vi "Periodic Log Filter Check.vi"(0 "Cross CSM Data":T2={"Name (\"\" to Use UUID)"="CSM Tiny", "Current State"="UI: Refresh Buttons", "Arguments"="", "Source Message"={"‘State"="", "’Arguments"="", "’Error"={"status"=FALSE, "code"=0, "source"=""}}, "Source Module"="<end>", "Complete(T)/Start(F)"=TRUE, "LogType"=enum."State Change", "Time Stamp"=timestamp(0 s since 1904-01-01)}, 1 "Reset?":bool, 9 "Remove Immediately? (F)":bool, 11 "Settings":T5={"threashold(#/s)"=2.0, "Check Peroid(s)"=1.0}, 12 "Level (Normal)":T1) -> (4 "Cross CSM Data Out":T2={"Name (\"\" to Use UUID)"="", "Current State"="", "Arguments"="", "Source Message"={"‘State"="", "’Arguments"="", "’Error"={"status"=FALSE, "code"=0, "source"=""}}, "Source Module"="", "Complete(T)/Start(F)"=FALSE, "LogType"=enum."State Change", "Time Stamp"=timestamp(0 s since 1904-01-01)}, 6 "Current Time":timestamp, 10 "Additional Info":string[](array[string]), 14 "Filtered Status":string[](array[string]), 15 "Filtered":bool)   [LabVIEW 2017, in "Communicable State Machine.lvlib" / "LogFilter.lvclass"]
uses:
  LogFilter.lvclass
  Typedef/_CSM_GlobalLog_MSG.ctl
  Typedef/_CSM_Response Source Message.ctl
  Typedef/_CSM_GlobalLog_MSG_TYPE.ctl
  Utility/_support/Periodic String Filter Level.ctl
  Utility/Periodic String Filter State.ctl
  Communicable State Machine.lvlib
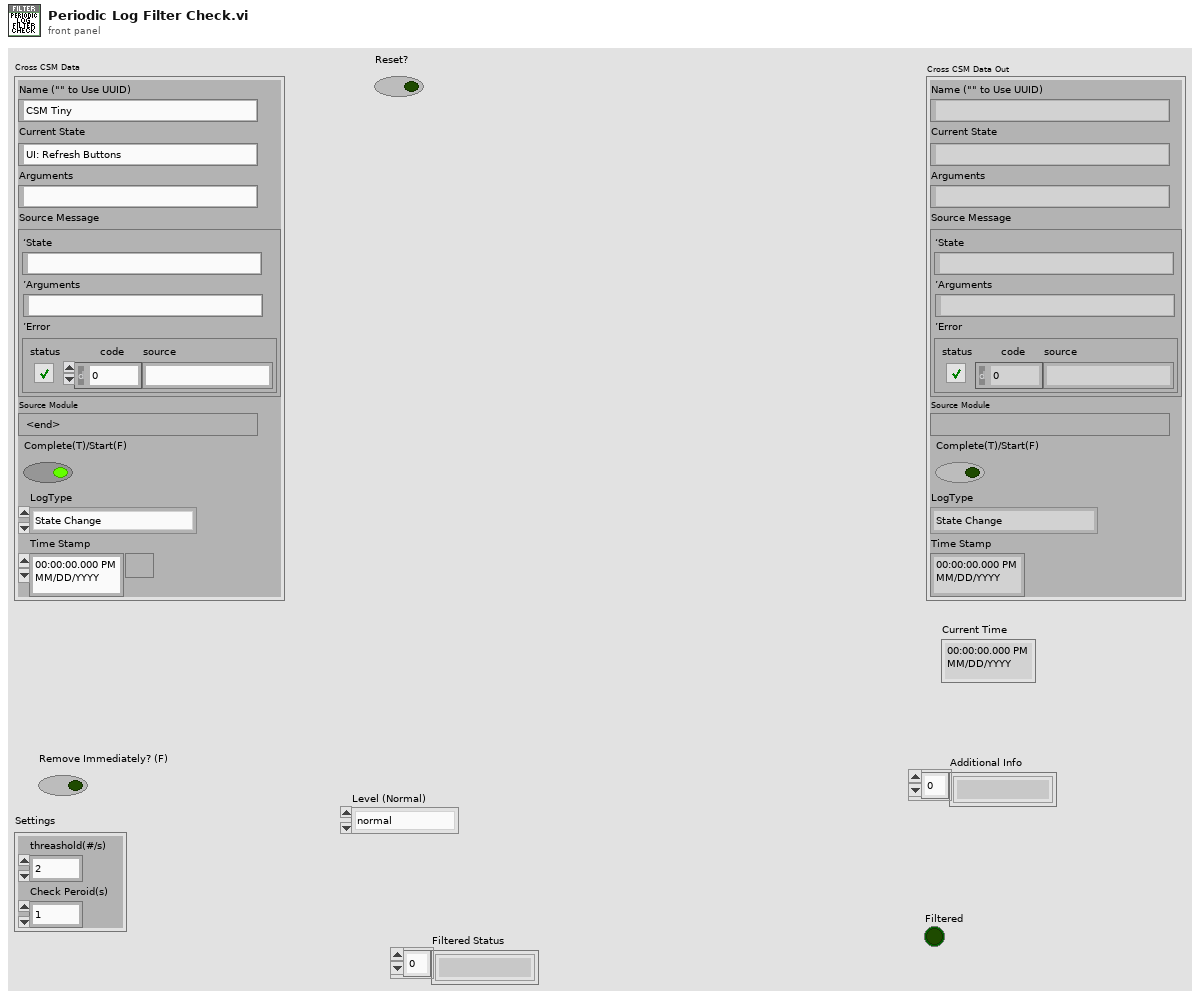
[diagram p1: front panel]
types:
  T1 = typedef "Communicable State Machine.lvlib/Periodic String Filter Level.ctl" = enum16{"normal", "L1", "L2", "L3", "L4"}
  T2 = typedef "Communicable State Machine.lvlib/_CSM_GlobalLog_MSG.ctl" = cluster{"Name (\"\" to Use UUID)":string, "Current State":string, "Arguments":string, "Source Message":T3, "Source Module":string, "Complete(T)/Start(F)":bool, "LogType":T4, "Time Stamp":timestamp}
  T3 = typedef "Communicable State Machine.lvlib/_CSM_Response Source Message.ctl" = cluster{"‘State":string, "’Arguments":string, "’Error":errorcluster}
  T4 = typedef "Communicable State Machine.lvlib/_CSM_GlobalLog_MSG_TYPE.ctl" = enum16{"User Log", "State Change", "Status", "Interrupt", "Register", "Unregister", "Error Log", "Module Created", "Module Destroyed"}
  T5 = cluster{"threashold(#/s)":dbl, "Check Peroid(s)":dbl}
  T6 = typedef "Communicable State Machine.lvlib/Periodic String Filter State.ctl" = enum16{"Normal", "Remove All Filters"}
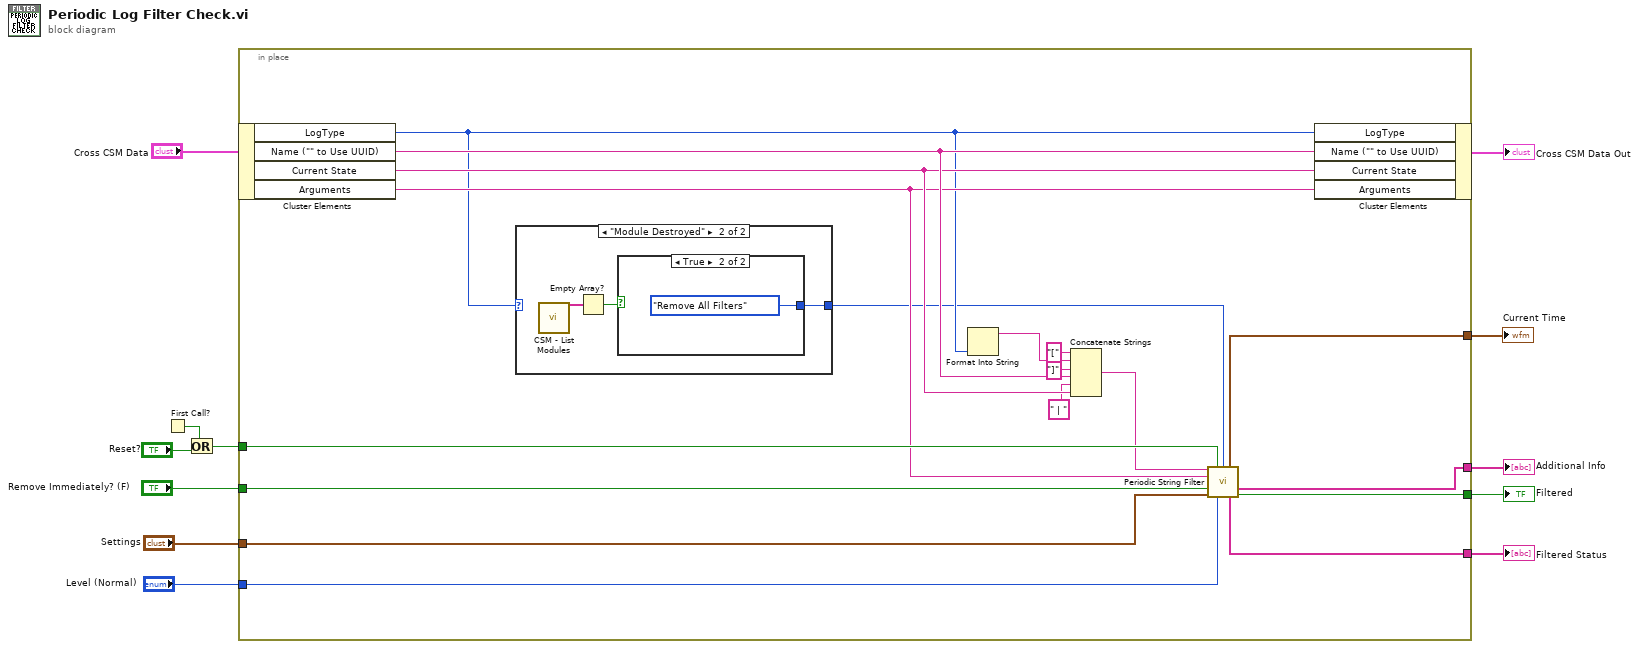
[diagram p0: block diagram]
diagram:
  n1 = First Call?() -> (First Call?: T/F=w11:bool)
  n2 = Or(x=w11, y="Reset?") -> (x .or. y?=w9:bool)
  n3 = in-place {
    in-place-border: w9 -> [w27]
    in-place-border: [w25] -> w8
    in-place-border: "Remove Immediately? (F)" -> [w22]
    in-place-border: "Settings" -> [w21]
    in-place-border: [w20] -> w1
    in-place-border: [w19] -> w4
    in-place-border: "Level (Normal)" -> [w16]
    in-place-border: [w15] -> w2
    n4 = in-place-cluster #1("Cross CSM Data") -> ("LogType"=w14:T4, "Name (\"\" to Use UUID)"=w30:string, "Current State"=w29:string, "Arguments"=w18:string)
    n5 = case shown="\"Module Destroyed\"" w14 {
      tunnel: [_ w31] -> w13
      frame "User Log", Default {
      }
      frame "Module Destroyed" {
        n6 = call "CSM - List Modules.vi"() -> ("Module Names"=w33:string[])  [unwired: 10 in, 1 out]
        n7 = Empty Array?(array=w33) -> (empty?=w32:bool)
        n8 = case shown="True" w32 {
          tunnel: [_ Periodic_String_Filter_State."Remove All Filters" ("State")] -> w31
          frame False {
          }
          frame True {
          }
        }
      }
    }
    n9 = Format Into String(w14) -> (resulting string=w17:string)  [unwired: 3 in, 1 out]
    n10 = Concatenate Strings("[" ("string"), w17, "]" ("string"), w30, " | " ("string"), w29) -> (w26:string)
    n11 = call "Periodic String Filter.vi"("Input String"=w26, "Reset?"=w27, "State"=w13, "Parameter"=w18, "Remove Immediately? (F)"=w22, "Settings"=w21, "Level (Normal)"=w16) -> ("Current Time"=w15:timestamp, "Additional Info"=w19:string[], "Filtered Status"=w20:string[], "Filtered?"=w25:bool)  [unwired: 4 in, 1 out]
    n12 = in-place-cluster #1("LogType"=w14, "Name (\"\" to Use UUID)"=w30, "Current State"=w29, "Arguments"=w18) -> (→"Cross CSM Data Out":T2)
  }
  "Filtered" <- w8
  "Filtered Status" <- w1
  "Additional Info" <- w4
  "Current Time" <- w2
